vi "Get File SFTP.vi"(8 "error in (no error)":errorcluster, 9 "local file path":path, 10 "remote path":string, 11 "session in":refnum<class "Session.lvclass">) -> (0 "error out":errorcluster, 3 "session out":refnum<class "Session.lvclass">)   [LabVIEW 2027, in "VeriStandTestUtilities.lvlib"]
uses:
  <vilib>/net/SFTP/Session/Session.lvclass
  <vilib>/net/SFTP/API/Download File.vi
  VeriStandTestUtilities.lvlib
  <vilib>/net/SFTP/NI_SFTP.lvlib
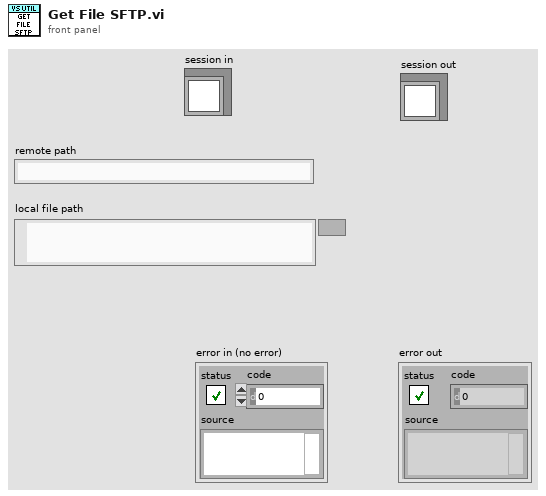
[diagram p1: front panel]
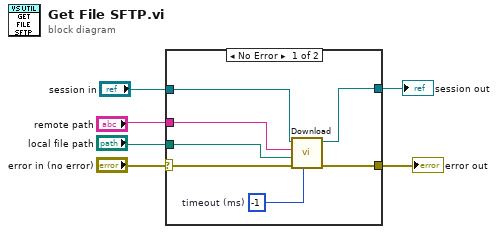
[diagram p0: block diagram]
diagram:
  n1 = case shown="No Error" "error in (no error)" {
    selector: "error in (no error)" -> [w13 w15]
    tunnel: [w12 w15] -> w5
    tunnel: "remote path" -> [w11 _]
    tunnel: "local file path" -> [w10 _]
    tunnel: "session in" -> [w8 w14]
    tunnel: [w7 w14] -> w1
    frame No Error {
      w9 = -1  # timeout (ms)
      n2 = call-poly <vilib>:"Download.vi"("timeout (ms)"=w9, "error in"=w13, "local path"=w10, "remote path"=w11, "session in"=w8) -> ("error out"=w12:errorcluster, "session out"=w7:refnum<class "Session.lvclass">)  [unwired: 5 in]
    }
    frame Error {
    }
  }
  "error out" <- w5
  "session out" <- w1
